vi "Show DBL postfix.vi"() -> ()   [LabVIEW 2017]
uses:
  c60d8553-bccd-48e7-aff5-5077e0d51e33.vi
  a74f769d-2f81-453e-8312-a8192043767a.vi
  0830f7fa-dccb-4097-ab6b-3c053261c739.vi
  3ade8e53-d78b-4aa0-b076-b259e10e2743.vi
  addons/API-String-Arugments-Support/_Support/Data To API String Arguments.vi
  addons/API-String-Arugments-Support/_Support/Convert API String Arguments to Data(variant).vi
panel:
  out "Array 6":dbl[](array[numeric])
  out "Array 5":dbl[](array[numeric])
  out "Array 4":string[](array[string])
  out "Array 3":string[](array[string])
  out "Array 2":string[](array[string])
  out "Array":string[](array[string])
  out "resulting string":string
  in  "input 1":dbl format="%#_15p"
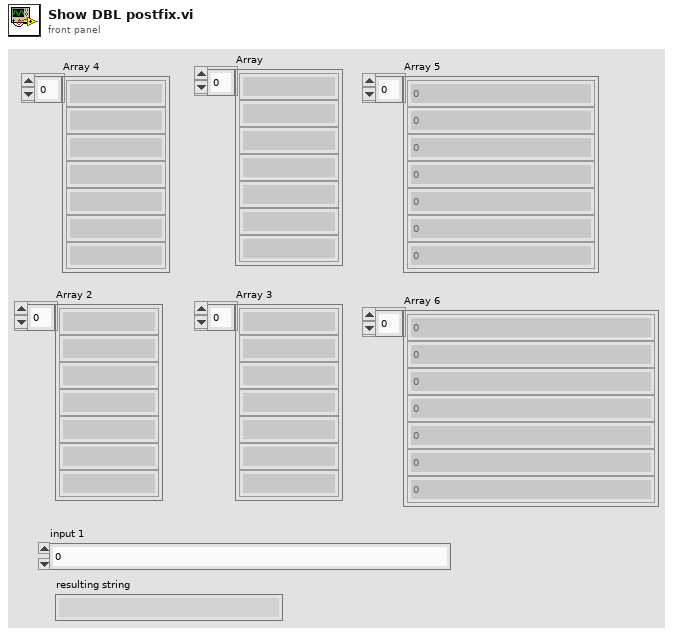
[diagram p1: front panel]
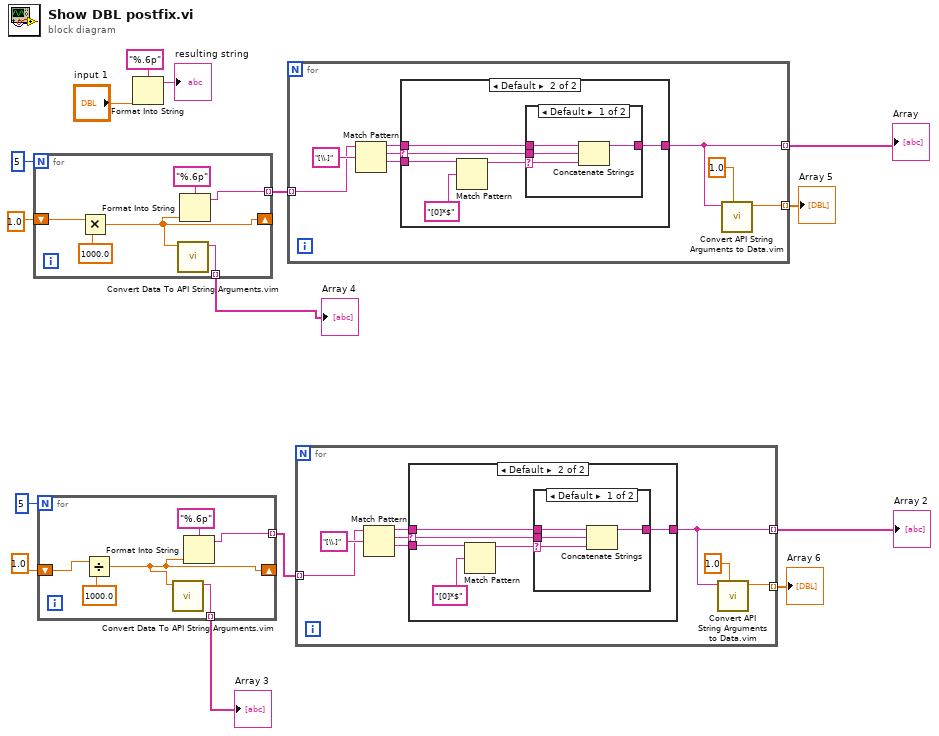
[diagram p0: block diagram]
diagram:
  n1 = for {
    N: 5 -> [_]
    shift-right: [w17] -> _
    shift-left: 1.0 ("input 2") -> [w21]
    tunnel: [w18] -> w8 mode=indexing
    tunnel: [w16] -> w3 mode=indexing
    n2 = Multiply(x=w21, y=1000.0) -> (x*y=w17:dbl)
    n3 = call "Convert Data To API String Arguments.vim"("data"=w17) -> ("String"=w16:string)  [unwired: 7 in, 1 out]
    n4 = Format Into String(format string="%.6p", w17) -> (resulting string=w18:string)  [unwired: 2 in, 1 out]
  }
  "Array 4" <- w3
  n5 = for {
    N: 5 -> [_]
    shift-right: [w23] -> _
    shift-left: 1.0 ("input 2") -> [w27]
    tunnel: [w24] -> w6 mode=indexing
    tunnel: [w22] -> w4 mode=indexing
    n6 = Divide(x=w27, y=1000.0) -> (x/y=w23:dbl)
    n7 = call "Convert Data To API String Arguments.vim"("data"=w23) -> ("String"=w22:string)  [unwired: 7 in, 1 out]
    n8 = Format Into String(format string="%.6p", w23) -> (resulting string=w24:string)  [unwired: 2 in, 1 out]
  }
  "Array 3" <- w4
  n9 = Format Into String(format string="%.6p", "input 1") -> (resulting string=→"resulting string":string)  [unwired: 2 in, 1 out]
  n10 = for {
    tunnel: w8 -> [w31] mode=indexing
    tunnel: [w30] -> w7 mode=indexing
    tunnel: [w28] -> w2 mode=indexing
    n11 = Match Pattern(string=w31, regular expression="[\\.]") -> (before substring=w33:string, match substring=w32:string, after substring=w34:string)  [unwired: 1 in, 1 out]
    n12 = case shown="Default" w32 {
      selector: w32 -> [_ w39]
      tunnel: w34 -> [_ w42]
      tunnel: w33 -> [w36 w40]
      tunnel: [w36 w37] -> w30
      frame "" {
      }
      frame Default {
        n13 = Match Pattern(string=w42, regular expression="[0]*$") -> (before substring=w38:string)  [unwired: 1 in, 3 out]
        n14 = case shown="Default" w38 {
          selector: w38 -> [w44 _]
          tunnel: w40 -> [w46 w47]
          tunnel: w39 -> [w45 _]
          tunnel: [w43 w47] -> w37
          frame Default {
            n15 = Concatenate Strings(w46, w45, w44) -> (w43:string)
          }
          frame "" {
          }
        }
      }
    }
    n16 = call "Convert API String Arguments to Data.vim"("Type"=1.0 ("input 2"), "String"=w30) -> ("Data"=w28:dbl)  [unwired: 6 in, 1 out]
  }
  "Array" <- w7
  "Array 5" <- w2
  n17 = for {
    tunnel: w6 -> [w51] mode=indexing
    tunnel: [w49] -> w5 mode=indexing
    tunnel: [w48] -> w1 mode=indexing
    n18 = Match Pattern(string=w51, regular expression="[\\.]") -> (before substring=w53:string, match substring=w52:string, after substring=w54:string)  [unwired: 1 in, 1 out]
    n19 = case shown="Default" w52 {
      selector: w52 -> [_ w59]
      tunnel: w54 -> [_ w62]
      tunnel: w53 -> [w56 w60]
      tunnel: [w56 w57] -> w49
      frame "" {
      }
      frame Default {
        n20 = Match Pattern(string=w62, regular expression="[0]*$") -> (before substring=w58:string)  [unwired: 1 in, 3 out]
        n21 = case shown="Default" w58 {
          selector: w58 -> [w64 _]
          tunnel: w60 -> [w66 w67]
          tunnel: w59 -> [w65 _]
          tunnel: [w63 w67] -> w57
          frame Default {
            n22 = Concatenate Strings(w66, w65, w64) -> (w63:string)
          }
          frame "" {
          }
        }
      }
    }
    n23 = call "Convert API String Arguments to Data.vim"("Type"=1.0 ("input 2"), "String"=w49) -> ("Data"=w48:dbl)  [unwired: 6 in, 1 out]
  }
  "Array 2" <- w5
  "Array 6" <- w1
